vi "Multi-mode acquisition.vi"() -> ()   [LabVIEW 2015]
doc: "Acquires sequences from the Andor iXon camera into Glimpse. \"Multi-mode\" means that the VI can be configured to sequentially acquire frames in multiple modes with different light sources and numbers of frames in each mode. Each mode is collected into a separate aquisition directory in Glimpse. Acquisition can be time-lapsed with a settable delay interval between cycles; the selected laser(s) are shuttered whilst not acquiring. The ixon setup acquisition.vi front panel is displayed so that the user can set the acquisition parameters before acquiring.\n\nThis is a Glimpse plug-in. To insure proper operation, you should have the source version of Glimpse running before loading this program. (The source version has an .llb extension, not a .exe one)."
uses:
  h-nu-ixon/Laser type.ctt
  h-nu-ixon/Emission filters.ctl
  ixon ultra1024/HAL camera parameters important.ctt
  ixon ultra1024/ixon readout settings.ctl
  ixon ultra1024/andor acquisition mode.ctl
  Glimpse core/Video acquisition state.ctl
  <vilib>/vision/Image Controls.llb/IMAQ Image.ctl
  Glimpse core/Seq file v 1/Offset table.ctl
  Glimpse core/Seq file v 1/Offset.ctl
  Glimpse core/Seq file v 1/file number.ctl
  ixon ultra1024/camera defaults globals.vi
  Stage/stage step to next field globals.vi
  Camera/camera globals.vi
  Glimpse core/GLIMPSE Globals.vi
  Autofocus Globals.vi
  h-nu-ixon/stage globals.vi
panel:
  in  "Max. number of acquisition files":i8(slide)=10 scale=0.0..50.0
  in  "Go? (F)":bool
  in  "Quit":bool
  in  "Delay after\nfilter change\n(ms)":u32
  in  "Scan fields options":T1(radio)
  in  "Scan Fields":bool
  in  "Max. cycles":i32=9999999
  in  "Cycle Interval (s)":dbl format="%_3f"
  in  "Camera Parameters":T2={"Exposure Time (sec)"=1.0, "EM CCD Gain"=230, "Readout Settings"={"Acquisition Mode"=enum."Frame Transfer Run till Abort", "Pixel Rate"=enum."EM CCD 20 Mhz 16 bits", "High Capacity?"=FALSE, "V Shift Speed (us/row)"=enum."4.33", "V Shift Amplitude"=enum."+1", "Preamp Gain"=enum."2", "Trigger Mode"=0, "Baseline offset"=0, "Baseline clamp"=TRUE}, "Image Size"={"H Bin"=1, "V Bin"=1, "Left"=1, "Top"=196, "Right"=1024, "Bottom"=730}} {"Readout Settings"."Baseline offset" min=-1000 max=1000 step=100; "Readout Settings"."Trigger Mode" items=["Internal", "External"]; "EM CCD Gain" scale=1.0..300.0; "Exposure Time (sec)" scale=0.001..10.0 scale format="%#_1g"}
  in  "Acquisition Protocol":T7(array[cluster]) {"Skip except for every Nth cycle, where N =" min=1 step=1; "Wait after frames (s)" format="%_3f"}
  # "Note:  In all panels, Ctrl-H displays the Context Help Window.  Hover mouse over panel icon or controls for context help."
  # "Camera: Andor iXon Ultra"
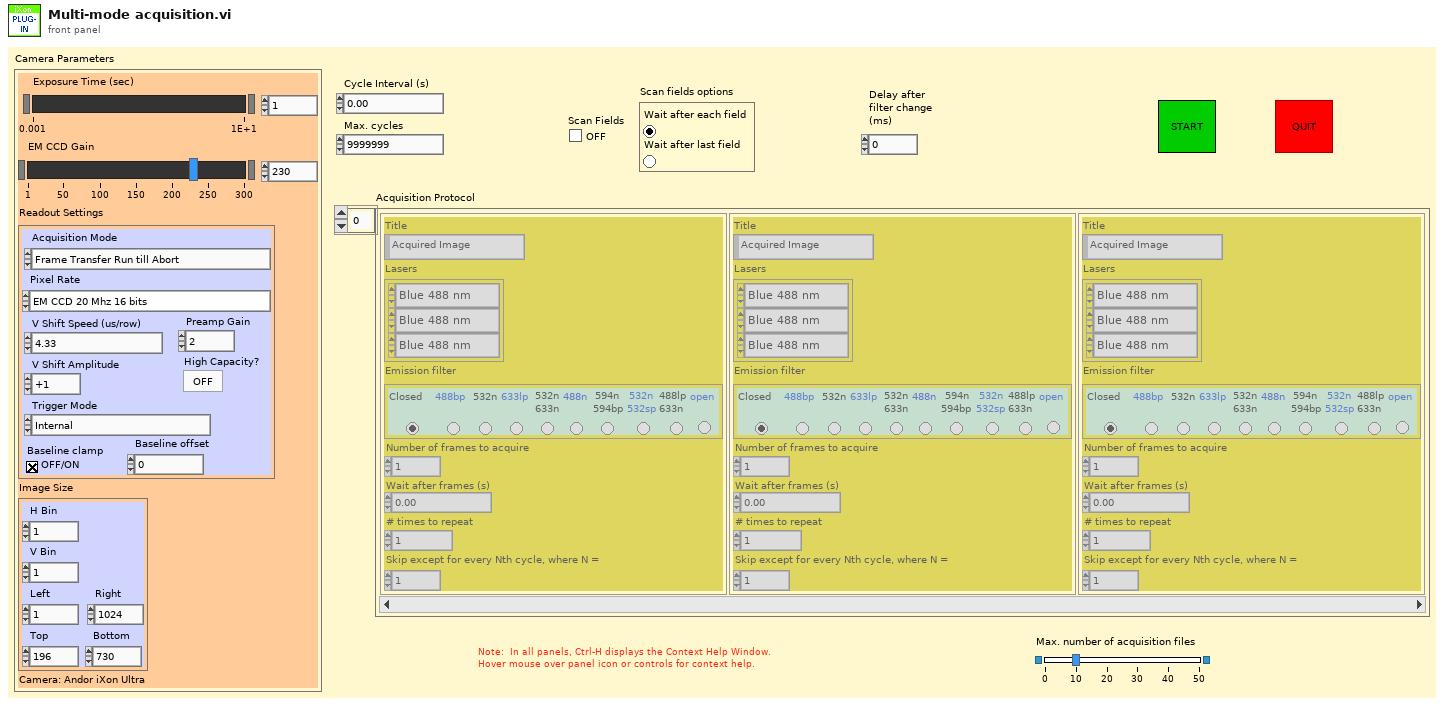
[diagram p1: front panel]
types:
  T1 = enum32{"Wait after each field", "Wait after last field"}
  T2 = typedef "HAL camera parameters important.ctt" = cluster{"Exposure Time (sec)":sgl, "EM CCD Gain":u16, "Readout Settings":T3, "Image Size":cluster{"H Bin":i32, "V Bin":i32, "Left":i32, "Top":i32, "Right":i32, "Bottom":i32}}
  T3 = typedef "ixon readout settings.ctl" = cluster{"Acquisition Mode":T4, "Pixel Rate":enum16{"EM CCD 30 Mhz 16 bits", "EM CCD 20 Mhz 16 bits", "EM CCD 10 Mhz 16 bits", "EM CCD 1 Mhz 16 bits", "Standard CCD 1 Mhz 16 bits", "Standard CCD 0.1 Mhz 16 bits"}, "High Capacity?":bool, "V Shift Speed (us/row)":enum16{"0.6", "1.13 ", "2.2 ", "4.33"}, "V Shift Amplitude":enum16{"normal", "+1", "+2", "+3", "+4"}, "Preamp Gain":enum16{"1", "2", "3"}, "Trigger Mode":u32, "Baseline offset":i16, "Baseline clamp":bool}
  T4 = typedef "andor acquisition mode.ctl" = enum16{"(do not use)", "Single Scan", "Accumulate", "Kinetics", "Fast Kinetics", "Kinetics Run till Abort", "Frame Transfer", "Frame Transfer Run till Abort", "(do not use) ", "Time Delayed Integration"}
  T5 = typedef "Laser type.ctt" = enum16{"Blue 488 nm", "Green 532 nm", "Orange 594 nm", "Red 633 nm", "IR 780"}
  T6 = typedef "Emission filters.ctl" = enum32{" Closed ", "488bp ", "532n", "633lp ", "532n\n633n", "488n", "594n\n594bp", "532n\n532sp", "488lp\n633n", "open"}
  T7 = cluster{"Title":string, "Lasers":T5[], "Emission filter":T6, "Number of frames to acquire":i32, "Wait after frames (s)":dbl, "# times to repeat":i32, "Skip except for every Nth cycle, where N =":i16}[]
  T8 = enum32{"None", "Manual", "Auto - Image analysis", "Auto - Retro-reflection"}
  T9 = typedef "image size.ctl" = cluster{"H Bin":i32, "V Bin":i32, "Left":i32, "Top":i32, "Right":i32, "Bottom":i32}
  T10 = typedef "Glimpse file parameters.ctt" = cluster{"Frame Size (bytes)":u32, "Max Frames":u32, "Max time (s)":u32, "Max Time (min)":u32, "Max Space Req'd. (Gb)":dbl, "Frames per acquisition file":u32}
  T11 = typedef "Video acquisition state.ctl" = cluster{"Pixel depth":enum32{"8 bits", "16 bits", "Float", "Complex", "RGB Chunky", "Compressed"}, "Width":dbl, "Height":dbl, "Buffer":T12, "Frames Acquired":u32, "Time of 1st frame":dbl, "TTB element zero":u32, "File Offsets Array":T13, "TTB Array":u32[], "Sum Image (for averaging)":T12, "Time at end of last acquisition (ms)":u32, "Filter array":u16[], "Flow rate array":dbl[], "Temperature array":dbl[], "Field array":u16[], "Lasers array":u16[][], "Stage xyz array":dbl[][]}
  T12 = typedef "IMAQ Image.ctl" = refnum<image>
  T13 = typedef "Offset table.ctl" = cluster{"offset":T14, "file number":T15}[]
  T14 = typedef "Offset.ctl" = i32
  T15 = typedef "file number.ctl" = u8
  T16 = typedef "Sequence files handle.ctt" = cluster{"Sequence files directory path":path, "Sequence files refnum array":refnum<file>[]}
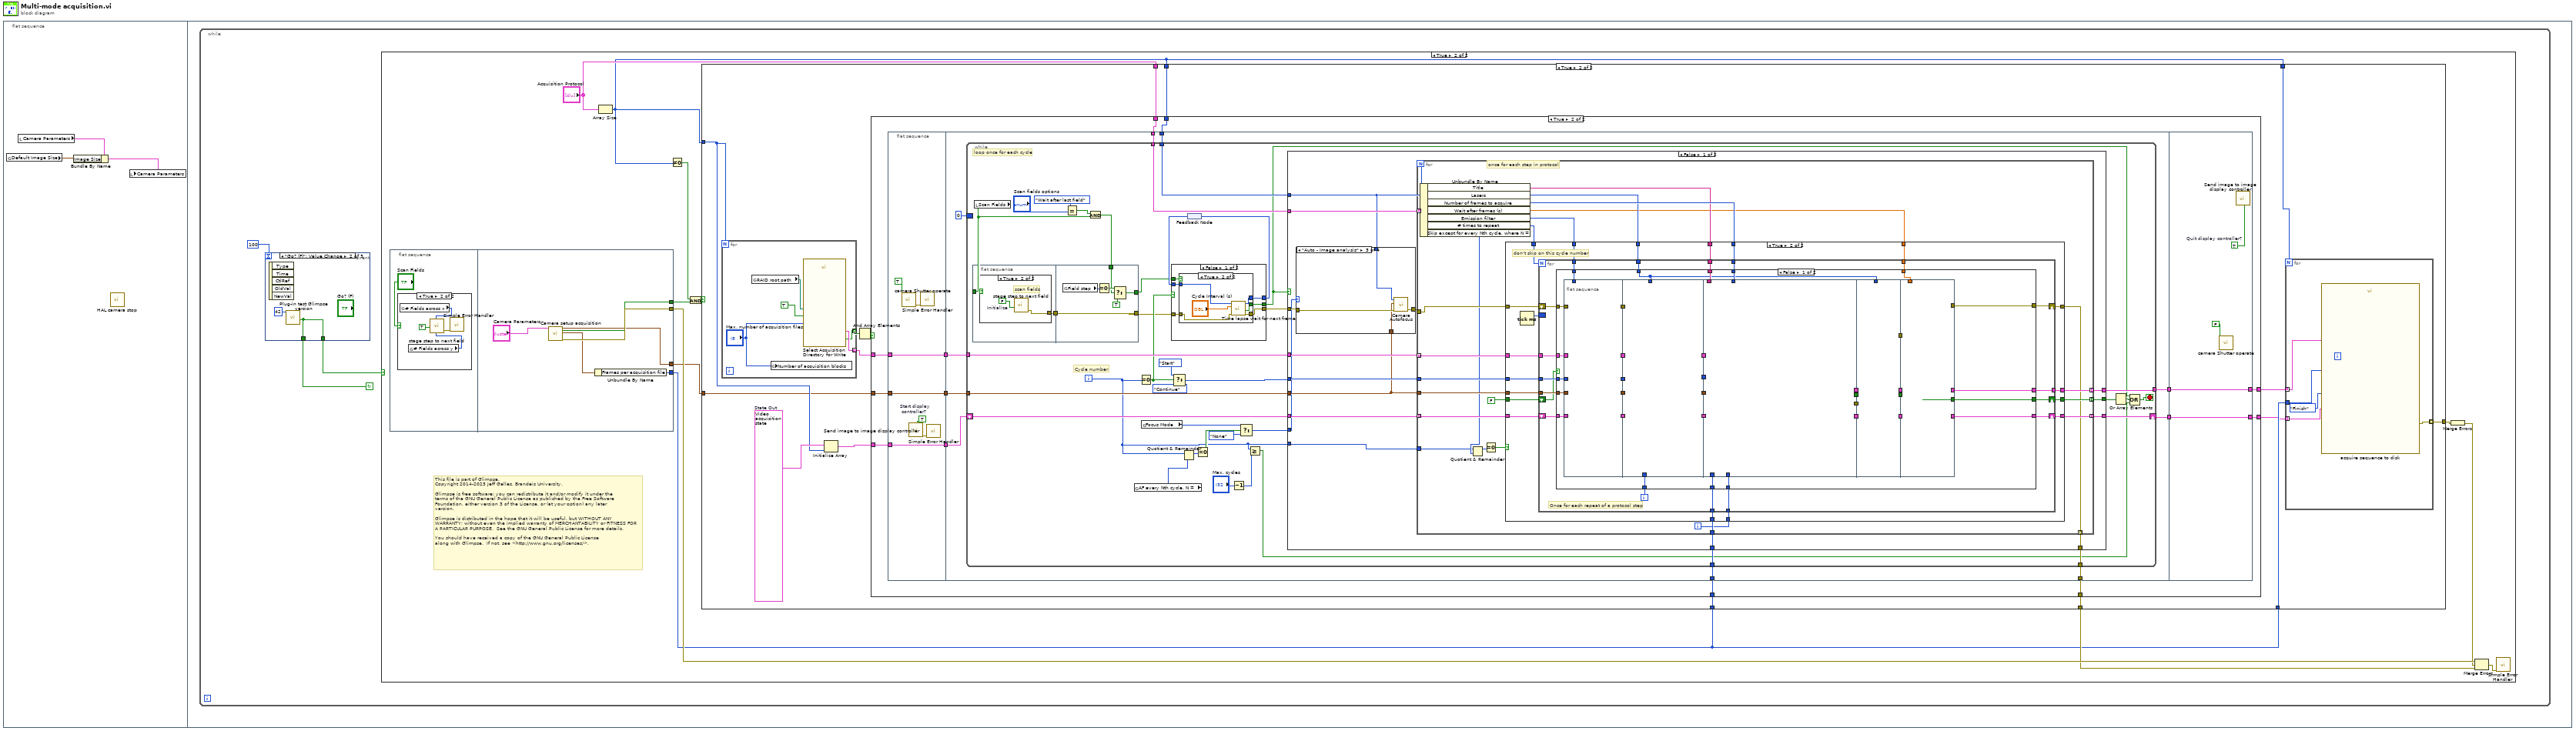
[diagram p0: block diagram]
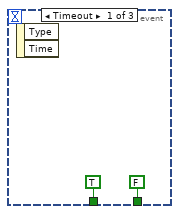
[diagram p2: hidden frame]
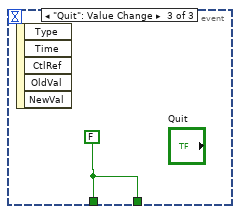
[diagram p3: hidden frame]
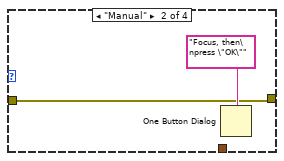
[diagram p9: hidden frame]
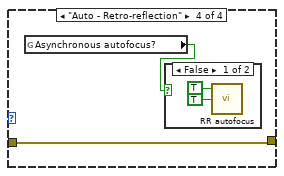
[diagram p10: hidden frame]
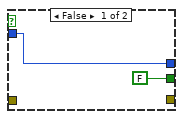
[diagram p16: hidden frame]
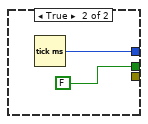
[diagram p17: hidden frame]
diagram:
  n1 = flat-sequence {
    frame #0 {
      n2 = global read "camera defaults globals.vi" "Default Image Size"() -> (w3:T9)
      n3 = local read "Camera Parameters"() -> (w2:T2)
      n4 = Bundle By Name(cluster=w2, "Image Size"=w3) -> (w1:T2)
      n5 = call "HAL camera stop.vi"() -> ()  [unwired: 1 in]
      n6 = local write "Camera Parameters"(w1) -> ()
    }
    frame #1 {
      n7 = while {
        stop <- w5 continue-if-true
        n8 = event shown="[1] \"Go? (F)\": Value Change" {
          selector: _ -> [_ _ _]
          dyn-events: _ -> [_ _ _]
          timeout: 100 -> [_ _ _]
          tunnel: [TRUE ("OK?") w9 w11] -> w5
          tunnel: [FALSE ("OK?") w9 w11] -> w4
          event Timeout {
            n9 = event-data() -> ()  [unwired: 1 in, 2 out]
          }
          event "Go? (F)": Value Change {
            n10 = event-data() -> ()  [unwired: 1 in, 5 out]
            n11 = call "Plug-in test Glimpse version.vi"("Minimum version required"=42) -> ("OK?"=w9:bool)  [unwired: 6 out]
          }
          event "Quit": Value Change {
            w11 = FALSE ("OK?")
            n12 = event-data() -> ()  [unwired: 1 in, 5 out]
          }
        }
        n13 = case shown="True" w4 {
          frame False {
          }
          frame True {
            # "This file is part of Glimpse. \nCopyright 2014-2023 Jeff Gelles, Brandeis University.    \n\nGlimpse is free software: you can redistribute it and/or modify it under the \nterms of the GNU General Public License as published by the Free Software \nFoundation, either version 3 of the License, or (at your option) any later \nversion.\n\nGlimpse is distributed in the hope that it will be useful, but WITHOUT ANY \nWARRANTY; without even the implied warranty of MERCHANTABILITY or FITNESS FOR \nA PARTICULAR PURPOSE.  See the GNU General Public License for more details.\n\nYou should have received a copy of the GNU General Public License\nalong with Glimpse.  If not, see <http://www.gnu.org/licenses/>."
            n14 = flat-sequence {
              tunnel: [w34] -> w23
              tunnel: [w33] -> w17
              tunnel: [w32] -> w14
              tunnel: [w29] -> w12
              frame #0 {
                n15 = case shown="True" "Scan Fields" {
                  frame False {
                  }
                  frame True {
                    n16 = global read "stage step to next field globals.vi" "# Fields across x"() -> (w26:i8)
                    n17 = global read "stage step to next field globals.vi" "# Fields across y"() -> (w25:i8)
                    n18 = call "stage step to next field.vi"("# Fields across x"=w26, "Initialize"=TRUE, "# Fields across y"=w25) -> ("error out"=w28:errorcluster)  [unwired: 2 in, 3 out]
                    n19 = call <vilib>:"Simple Error Handler.vi"("error in (no error)"=w28) -> ()  [unwired: 1 in, 8 out]
                  }
                }
              }
              frame #1 {
                n20 = call "Camera setup acquisition.vi"("Camera Parameters (important)"="Camera Parameters") -> ("Image Size Out"=w32:T9, "Continue with acq?"=w33:bool, "Glimpse file properties"=w30:T10, "Error Out (no error)"=w34:errorcluster)  [unwired: 6 in, 9 out]
                n21 = Unbundle By Name(w30) -> ("Frames per acquisition file"=w29:u32)
              }
            }
            n22 = Array Size(array="Acquisition Protocol") -> (size(s)=w16:i32)
            n23 = Not Equal To 0?(x=w16) -> (x != 0?=w15:bool)
            n24 = And(x=w15, y=w17) -> (x .and. y?=w18:bool)
            n25 = case shown="True" w18 {
              tunnel: w12 -> [_ w49]
              tunnel: w12 -> [_ w48]
              tunnel: [_ w47] -> w21
              tunnel: [_ w46] -> w22
              tunnel: w16 -> [_ w36]
              tunnel: w16 -> [_ w42]
              tunnel: w16 -> [_ w39]
              tunnel: "Acquisition Protocol" -> [_ w37]
              tunnel: w14 -> [_ w35]
              frame False {
              }
              frame True {
                w41 = T11 {"Pixel depth"=enum."8 bits", "Width"=0.0, "Height"=0.0, "Buffer"=refnum, "Frames Acquired"=0, "Time of 1st frame"=0.0, "TTB element zero"=0, "File Offsets Array"=[], "TTB Array"=[], "Sum Image (for averaging)"=refnum, "Time at end of last acquisition (ms)"=0, "Filter array"=[], "Flow rate array"=[], "Temperature array"=[], "Field array"=[], "Lasers array"=[], "Stage xyz array"=[]}  # State Out
                n26 = for {
                  N: w36 -> [_]
                  tunnel: [w341] -> w38 mode=indexing
                  tunnel: [w340] -> w50 mode=indexing
                  n27 = global read "GLIMPSE Globals.vi" "RAID root path"() -> (w343:path)
                  n28 = global write "camera globals.vi" "Number of acquisition blocks"("Max. number of acquisition files") -> ()
                  n29 = call "Select Acquisition Directory for Write.vi"("Autostart?"=TRUE, "Acquisition directory root path"=w343, "Number of acquisition files"="Max. number of acquisition files") -> ("Sequence files handle"=w341:T16, "OK?"=w340:bool)  [unwired: 11 out]
                }
                n30 = Initialize Array(w41, w36) -> (w40:T11[])
                n31 = And Array Elements(Boolean array=w50) -> (logical AND=w43:bool)
                n32 = case shown="True" w43 {
                  tunnel: [w57 w72] -> w45
                  tunnel: w38 -> [w57 w71]
                  tunnel: w49 -> [_ w70]
                  tunnel: [w58 w69] -> w44
                  tunnel: [_ w68] -> w47
                  tunnel: w42 -> [_ w67]
                  tunnel: w40 -> [w58 w66]
                  tunnel: w37 -> [_ w65]
                  tunnel: w35 -> [_ w60]
                  frame False {
                  }
                  frame True {
                    n33 = flat-sequence {
                      tunnel: w66 -> [w78]
                      tunnel: w71 -> [w79]
                      tunnel: [w79] -> w64
                      tunnel: [w78] -> w63
                      tunnel: w60 -> [w76]
                      tunnel: [w76] -> w59
                      tunnel: w70 -> [w87]
                      tunnel: [w85] -> w68
                      tunnel: w67 -> [w84]
                      tunnel: w65 -> [w82]
                      tunnel: w64 -> [w88]
                      tunnel: w63 -> [w83]
                      tunnel: [w89] -> w62
                      tunnel: [w86] -> w61
                      tunnel: w59 -> [w81]
                      tunnel: [w337] -> w69
                      tunnel: [w338] -> w72
                      tunnel: w62 -> [w338]
                      tunnel: w61 -> [w337]
                      frame #0 {
                        w75 = TRUE  # Start display  controller?
                        n34 = call "camera Shutter operate.vi"("Open?"=TRUE) -> ("error out"=w73:errorcluster)  [unwired: 1 in, 6 out]
                        n35 = call "Send image to image display controller.vi"("Start display controller?"=w75) -> ("error out"=w74:errorcluster)  [unwired: 6 in, 3 out]
                        n36 = call <vilib>:"Simple Error Handler.vi"("error in (no error)"=w73) -> ()  [unwired: 1 in, 8 out]
                        n37 = call <vilib>:"Simple Error Handler.vi"("error in (no error)"=w74) -> ()  [unwired: 1 in, 8 out]
                      }
                      frame #1 {
                        n38 = while {
                          tunnel: [w127] -> w89
                          tunnel: w88 -> [w126]
                          tunnel: w87 -> [w125]
                          shift-right: [w123] -> w86
                          shift-left: w83 -> [w124]
                          tunnel: [w122] -> w85
                          tunnel: w84 -> [w110]
                          tunnel: w82 -> [w116]
                          tunnel: w81 -> [w111]
                          border: u32 0 -> [_]
                          i -> [w90]
                          stop <- w114 stop-if-true
                          # "Cycle number"
                          # "loop once for each cycle"
                          n39 = flat-sequence {
                            tunnel: w97 -> [w310]
                            tunnel: [w309] -> w98
                            tunnel: [w318] -> w103
                            tunnel: w98 -> [w318]
                            tunnel: w95 -> [w314]
                            tunnel: [w313] -> w96
                            frame #0 {
                              n40 = case shown="True" w310 {
                                tunnel: [_ w311] -> w309
                                frame False {
                                }
                                frame True {
                                w312 = FALSE  # Initialize
                                # "scan fields"
                                n41 = call "stage step to next field.vi"("Initialize"=w312) -> ("error out"=w311:errorcluster)  [unwired: 4 in, 3 out]
                                }
                              }
                            }
                            frame #1 {
                              n42 = global read "stage globals.vi" "Field step"() -> (w315:i16)
                              n43 = Equal To 0?(x=w315) -> (x = 0?=w316:bool)
                              n44 = Select(t=w316, s=w314, f=TRUE) -> (s? t:f=w313:bool)
                            }
                          }
                          n45 = local read "Scan Fields"() -> (w97:bool)
                          n46 = Equal?(x="Scan fields options", y=T1."Wait after last field") -> (x = y?=w94:bool)
                          n47 = And(x=w94, y=w97) -> (x .and. y?=w95:bool)
                          n48 = global read "Autofocus Globals.vi" "AF every Nth cycle, N ="() -> (w109:u8)
                          n49 = Equal To 0?(x=w90) -> (x = 0?=w115:bool)
                          n50 = global read "Autofocus Globals.vi" "Focus Mode"() -> (w101:T8)
                          n51 = Select(t=enum16{"Start", "Continue", "Finish"}."Start" ("Operation"), s=w115, f=enum16{"Start", "Continue", "Finish"}."Continue" ("Operation")) -> (s? t:f=w119:enum16{"Start", "Continue", "Finish"})
                          n52 = Quotient & Remainder(x=w90, y=w109) -> (x-y*floor(x/y)=w108:i32)  [unwired: 1 out]
                          n53 = feedback #1() -> (w112:u32)
                          n54 = case shown="False" w115 {
                            tunnel: [w324 w334] -> w113
                            tunnel: [w323 FALSE] -> w91
                            tunnel: w112 -> [w322 _]
                            tunnel: [w321 _] -> w104
                            tunnel: w96 -> [w320 _]
                            tunnel: w103 -> [w319 _]
                            frame False {
                              n55 = case shown="True" w320 {
                                tunnel: [w326 w332] -> w324
                                tunnel: [FALSE ("Stopped?") w331] -> w323
                                tunnel: w322 -> [w326 w330]
                                tunnel: [_ w328] -> w321
                                tunnel: w319 -> [_ w327]
                                frame False {
                                }
                                frame True {
                                n56 = call "Time lapse wait for next frame.vi"("error in (no error)"=w327, "Frame Interval (s)"="Cycle Interval (s)", "Time of last frame in"=w330) -> ("error out"=w328:errorcluster, "Stopped?"=w331:bool, "Time of this frame out (ms)"=w332:u32)  [unwired: 4 out]
                                }
                              }
                            }
                            frame True {
                              n57 = Tick Count (ms)() -> (millisecond timer value=w334:u32)
                            }
                          }
                          n58 = feedback-in #1(w113) -> ()
                          n59 = Equal To 0?(x=w108) -> (x = 0?=w102:bool)
                          n60 = Decrement(x="Max. cycles") -> (x-1=w105:i32)
                          n61 = Select(t=w101, s=w102, f=T8."None") -> (s? t:f=w99:T8)
                          n62 = Greater Or Equal?(x=w90, y=w105) -> (x >= y?=w106:bool)
                          n63 = case shown="False" w91 {
                            tunnel: [w142 w307] -> w127
                            tunnel: w126 -> [w141 w307]
                            tunnel: w125 -> [w140 _]
                            tunnel: w124 -> [w139 w308]
                            tunnel: [w138 w308] -> w123
                            tunnel: [w137 _] -> w122
                            tunnel: w119 -> [w136 _]
                            tunnel: [w135 _] -> w118
                            tunnel: w116 -> [w134 _]
                            tunnel: w111 -> [w132 _]
                            tunnel: w110 -> [w131 _]
                            tunnel: w104 -> [w130 _]
                            tunnel: w99 -> [w129 _]
                            tunnel: w90 -> [w128 _]
                            frame False {
                              n64 = case shown="\"Auto - Image analysis\"" w129 {
                                tunnel: w130 -> [w143 w144 w149 w151]
                                tunnel: [w143 w144 w148 w151] -> w133
                                tunnel: w132 -> [_ _ w147 _]
                                tunnel: w131 -> [_ _ w146 _]
                                frame "None", Default {
                                }
                                frame "Manual" {
                                n65 = One Button Dialog(message="Focus, then\npress \"OK\"") -> ()  [unwired: 2 out]
                                }
                                frame "Auto - Image analysis" {
                                n66 = call "Camera Autofocus.vi"("error in"=w149, "Image Size"=w147, "Display Window Number"=w146) -> ("error out"=w148:errorcluster)  [unwired: 2 in, 6 out]
                                }
                                frame "Auto - Retro-reflection" {
                                n67 = global read "Autofocus Globals.vi" "Asynchronous autofocus?"() -> (w150:bool)
                                n68 = case shown="False" w150 {
                                frame False {
                                n69 = call "RR autofocus.vi"("Close camera shutter during autofocus?"=TRUE, "Close laser shutter when autofocus is done?"=TRUE) -> ()  [unwired: 5 in, 1 out]
                                }
                                frame True {
                                }
                                }
                                }
                              }
                              n70 = for {
                                N: w131 -> [_]
                                tunnel: [w176] -> w142 mode=indexing
                                tunnel: w141 -> [w175] mode=indexing
                                tunnel: w140 -> [w174]
                                tunnel: w139 -> [w169] mode=indexing
                                tunnel: [w173] -> w138 mode=indexing
                                tunnel: [w172] -> w135 mode=indexing
                                tunnel: [w171] -> w137 mode=indexing
                                tunnel: w136 -> [w170]
                                tunnel: w134 -> [w168] mode=indexing
                                tunnel: w133 -> [w164]
                                tunnel: w132 -> [w163]
                                tunnel: w128 -> [w155]
                                i -> [w166]
                                # "once for each step in protocol"
                                n71 = Unbundle By Name(w168) -> ("Title"=w165:string, "Lasers"=w162:T5[], "Number of frames to acquire"=w167:i32, "Wait after frames (s)"=w161:dbl, "Emission filter"=w159:T6, "# times to repeat"=w160:i32, "Skip except for every Nth cycle, where N ="=w156:i16)
                                n72 = Quotient & Remainder(x=w155, y=w156) -> (x-y*floor(x/y)=w158:i32)  [unwired: 1 out]
                                n73 = Equal To 0?(x=w158) -> (x = 0?=w157:bool)
                                n74 = case shown="True" w157 {
                                tunnel: [w178 w199] -> w176
                                tunnel: w175 -> [w178 w198]
                                tunnel: w174 -> [_ w197]
                                tunnel: [w179 w196] -> w173
                                tunnel: [w177 w195] -> w172
                                tunnel: [w180 w194] -> w171
                                tunnel: w170 -> [_ w193]
                                tunnel: w169 -> [w179 w192]
                                tunnel: w167 -> [_ w191]
                                tunnel: w166 -> [_ w190]
                                tunnel: w165 -> [_ w189]
                                tunnel: w164 -> [w180 w188]
                                tunnel: w163 -> [_ w187]
                                tunnel: w162 -> [_ w186]
                                tunnel: w161 -> [_ w184]
                                tunnel: w160 -> [_ w183]
                                tunnel: w159 -> [_ w182]
                                tunnel: FALSE -> [w177 w181]
                                frame False {
                                # "skip on this cycle number"
                                }
                                frame True {
                                # "don't skip on this cycle number"
                                n75 = Tick Count (ms)() -> (millisecond timer value=w185:u32)
                                n76 = for {
                                N: w183 -> [_]
                                tunnel: [w217] -> w199
                                tunnel: w198 -> [w216]
                                tunnel: w197 -> [w215]
                                tunnel: w193 -> [w211]
                                tunnel: w191 -> [w209]
                                tunnel: w190 -> [w208]
                                tunnel: w189 -> [w207]
                                tunnel: w187 -> [w205]
                                tunnel: w186 -> [w204]
                                shift-right: [w214] -> w196
                                shift-left: w192 -> [w210]
                                border: w185 -> [_]
                                tunnel: w184 -> [w203]
                                shift-right: [w213] -> w195
                                shift-left: w181 -> [w202]
                                shift-right: [w212] -> w194
                                shift-left: w188 -> [w206]
                                tunnel: w182 -> [w200]
                                i -> [w201]
                                # "Once for each repeat of a protocol step"
                                n77 = case shown="False" w202 {
                                selector: w202 -> [_ w306]
                                tunnel: [w239 w303] -> w217
                                tunnel: w216 -> [w238 w303]
                                tunnel: w215 -> [w237 _]
                                tunnel: [w236 w305] -> w214
                                tunnel: [w235 w306] -> w213
                                tunnel: [w234 w304] -> w212
                                tunnel: w211 -> [w233 _]
                                tunnel: w210 -> [w232 w305]
                                tunnel: w209 -> [w231 _]
                                tunnel: w208 -> [w230 _]
                                tunnel: w207 -> [w229 _]
                                tunnel: w206 -> [w228 w304]
                                tunnel: w205 -> [w227 _]
                                tunnel: w204 -> [w226 _]
                                tunnel: w203 -> [w225 _]
                                tunnel: w201 -> [w224 _]
                                tunnel: w200 -> [w223 _]
                                frame False {
                                n78 = flat-sequence {
                                tunnel: w227 -> [w256]
                                tunnel: w228 -> [w254]
                                tunnel: w232 -> [w257]
                                tunnel: w233 -> [w258]
                                tunnel: w238 -> [w259]
                                tunnel: [w259] -> w222
                                tunnel: [w258] -> w221
                                tunnel: [w257] -> w220
                                tunnel: [w253] -> w219
                                tunnel: [w256] -> w218
                                tunnel: w223 -> [w255]
                                tunnel: [w271] -> w251
                                tunnel: w226 -> [w268]
                                tunnel: [w261] -> w250
                                tunnel: [w267] -> w249
                                tunnel: [w266] -> w248
                                tunnel: w224 -> [w263]
                                tunnel: w222 -> [w271]
                                tunnel: w221 -> [w262]
                                tunnel: w220 -> [w267]
                                tunnel: w219 -> [w260]
                                tunnel: w218 -> [w266]
                                tunnel: w251 -> [w273]
                                tunnel: [w274] -> w247
                                tunnel: [w272] -> w246
                                tunnel: [w275] -> w245
                                tunnel: w237 -> [w282]
                                tunnel: [w276] -> w244
                                tunnel: w250 -> [w279]
                                tunnel: w249 -> [w277]
                                tunnel: w231 -> [w280]
                                tunnel: w230 -> [w284]
                                tunnel: w229 -> [w283]
                                tunnel: w248 -> [w281]
                                tunnel: w247 -> [w291]
                                tunnel: [w291] -> w243
                                tunnel: w246 -> [w290]
                                tunnel: [w290] -> w242
                                tunnel: w245 -> [w286]
                                tunnel: w244 -> [w289]
                                tunnel: [w289] -> w241
                                tunnel: w226 -> [w287]
                                tunnel: [w285] -> w240
                                tunnel: [w301] -> w239
                                tunnel: [w302] -> w236
                                tunnel: w243 -> [w302]
                                tunnel: w242 -> [w301]
                                tunnel: w241 -> [w299]
                                tunnel: [w298] -> w235
                                tunnel: [w293] -> w234
                                tunnel: w225 -> [w295]
                                tunnel: w240 -> [w294]
                                frame #0 {
                                n79 = call "Select emission filter.vi"("Emission filter"=w255, "Time to wait\nafter filter change\n(ms)"="Delay after\nfilter change\n(ms)", "error in"=w254) -> ("error out"=w253:errorcluster)  [unwired: 3 out]
                                }
                                frame #1 {
                                n80 = Equal To 0?(x=w263) -> (x = 0?=w264:bool)
                                n81 = call "Shutter operate.vi"("Shutters"=w268, 2:TRUE ("Data to Write"), "error in"=w260) -> ("error out"=w269:errorcluster)  [unwired: 5 out]
                                n82 = call <vilib>:"Simple Error Handler.vi"("error in (no error)"=w269) -> ()  [unwired: 1 in, 8 out]
                                n83 = Select(t=w262, s=w264, f=enum16{"Start", "Continue", "Finish"}."Continue" ("Operation")) -> (s? t:f=w261:enum16{"Start", "Continue", "Finish"})
                                }
                                frame #2 {
                                n84 = call "acquire sequence to disk.vi"("Image Size"=w281, "State In"=w277, "Frames per acquisition file"=w282, "Sequence files handle"=w273, "Pressing stop automatically runs finish?"=FALSE, "Display Window Title"=w283, "Operation"=w279, "Display Window Number"=w284, "Number of frames to acquire"=w280) -> ("Done?"=w276:bool, "State Out"=w274:T11, "Sequence files handle out"=w272:T16, "error out"=w275:errorcluster)  [unwired: 2 in, 5 out]
                                }
                                frame #3 {
                                n85 = call "Shutter operate.vi"("Shutters"=w287, 2:FALSE ("Data to Write"), "error in"=w286) -> ("error out"=w285:errorcluster)  [unwired: 5 out]
                                }
                                frame #4 {
                                n86 = feedback #2() -> (w296:u32)
                                n87 = call "Time lapse wait for next frame.vi"("error in (no error)"=w294, "Frame Interval (s)"=w295, "Time of last frame in"=w296) -> ("error out"=w293:errorcluster, "Stopped?"=w292:bool, "Time of this frame out (ms)"=w297:u32)  [unwired: 4 out]
                                n88 = Unbundle By Name(w293) -> ("status"=w300:bool)
                                n89 = feedback-in #2(w297) -> ()
                                n90 = Compound Arithmetic op=OR(w292, w299, w300) -> (w298:bool)
                                }
                                }
                                }
                                frame True {
                                }
                                }
                                }
                                }
                                }
                              }
                            }
                            frame True {
                            }
                          }
                          n91 = Or Array Elements(Boolean array=w118) -> (logical OR=w117:bool)
                          n92 = Compound Arithmetic op=OR(w91, w117, w106) -> (w114:bool)
                        }
                      }
                      frame #2 {
                        w336 = TRUE  # Quit display controller?
                        n93 = call "camera Shutter operate.vi"("Open?"=FALSE) -> ()  [unwired: 1 in, 7 out]
                        n94 = call "Send image to image display controller.vi"("Quit display controller?"=w336) -> ()  [unwired: 6 in, 4 out]
                      }
                    }
                  }
                }
                n95 = for {
                  N: w39 -> [_]
                  tunnel: w48 -> [w54]
                  tunnel: [w51] -> w46 mode=indexing
                  tunnel: w45 -> [w56] mode=indexing
                  tunnel: w44 -> [w52] mode=indexing
                  i -> [w55]
                  n96 = call "acquire sequence to disk.vi"("State In"=w52, "Frames per acquisition file"=w54, "Sequence files handle"=w56, "Operation"=enum16{"Start", "Continue", "Finish"}."Finish", "Display Window Number"=w55) -> ("error out"=w51:errorcluster)  [unwired: 6 in, 8 out]
                }
              }
            }
            n97 = Merge Errors(w22) -> (w20:errorcluster)
            n98 = Merge Errors(w23, w20, w21) -> (w13:errorcluster)
            n99 = call <vilib>:"Simple Error Handler.vi"("error in (no error)"=w13) -> ()  [unwired: 1 in, 8 out]
          }
        }
      }
    }
  }
